vi "conf FCC Main Worst Position Measurement.vi"(8 "error in (no error)":errorcluster, 11 "SA Measurement in":refnum<class "SA Measurement.lvclass">) -> (0 "error out":errorcluster, 3 "SA Measurement out":refnum<class "SA Measurement.lvclass">)   [LabVIEW 2023, in "Spectrum Analyzer.lvlib" / "SA Measurement.lvclass"]
uses:
  SA Measurement.lvclass
  TYPE DEFINITION/Keysight 9020A/TYPE Measurement Preset.ctl
  TYPE DEFINITION/TYPE RBW and VBW Select.ctl
  TYPE DEFINITION/TYPE Marker Auto Select.ctl
  TYPE DEFINITION/TYPE Marker Control Mode.ctl
  SA Measurement.lvclass/SA Measurement.ctl
  Interface_Spectrum/Interface_Spectrum.lvclass
  Spectrum Analyzer.lvlib
  TYPE DEFINITION/TYPE Sweep Type Select.ctl
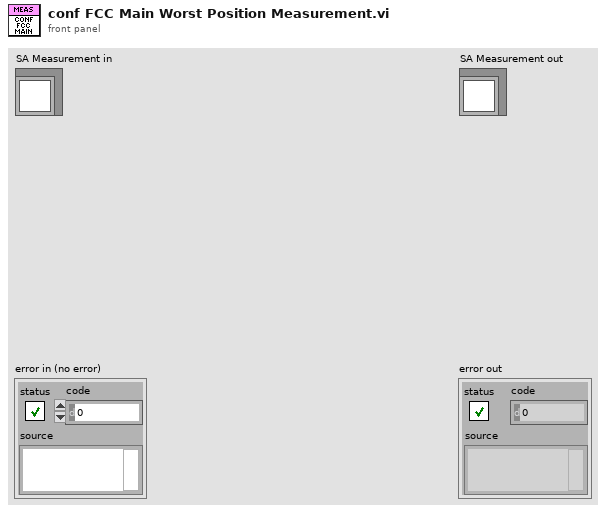
[diagram p1: front panel]
types:
  T1 = typedef "Spectrum Analyzer.lvlib/TYPE Sweep Type Select.ctl" = enum16{"Auto", "Sweep", "FFT"}
  T2 = typedef "Spectrum Analyzer.lvlib/TYPE Marker Control Mode.ctl" = enum16{"Normal", "Delta", "Off"}
  T3 = typedef "Spectrum Analyzer.lvlib/TYPE Marker Auto Select.ctl" = enum16{"Max Search Auto", "Min Search Auto"}
  T4 = typedef "Spectrum Analyzer.lvlib/TYPE RBW and VBW Select.ctl" = enum16{"Res BW", "Video BW"}
  T5 = typedef "Spectrum Analyzer.lvlib/TYPE Measurement Preset.ctl" = enum16{"Sweep SA Mode", "Channel Power", "Occupied BW", "ACP", "Spurious Emission", "Spurious Emission Mask", "Burst Power (Transmit Power)"}
  T6 = typedef "Spectrum Analyzer.lvlib/TYPE Y-axis Unit.ctl" = enum16{"dBm", "dBmV", "dBuV", "dBpW", "Volt", "Ampere", "Watt"}
  T7 = typedef "Spectrum Analyzer.lvlib/TYPE Reference Level and Atten Param.ctl" = cluster{"Reference Level":dbl, "Atten":i32, "Atten Auto?":bool, "Reference Level Offset":dbl}
  T8 = typedef "Spectrum Analyzer.lvlib/TYPE Display Trace Mode Select.ctl" = enum16{"Clear Write", "Max Hold", "Min Hold", "Average", "View"}
  T9 = typedef "Spectrum Analyzer.lvlib/TYPE Detect Mode Select.ctl" = enum16{"Det Auto (Normal)", "Auto Peak", "Positive Peak", "Negative Peak", "Sample", "RMS", "Average", "Quasipeak", "CISPR Average", "RMS Average"}
  T10 = cluster{"Trace Mode":T8, "Detector Type":T9, "Detect Auto?":bool}[]
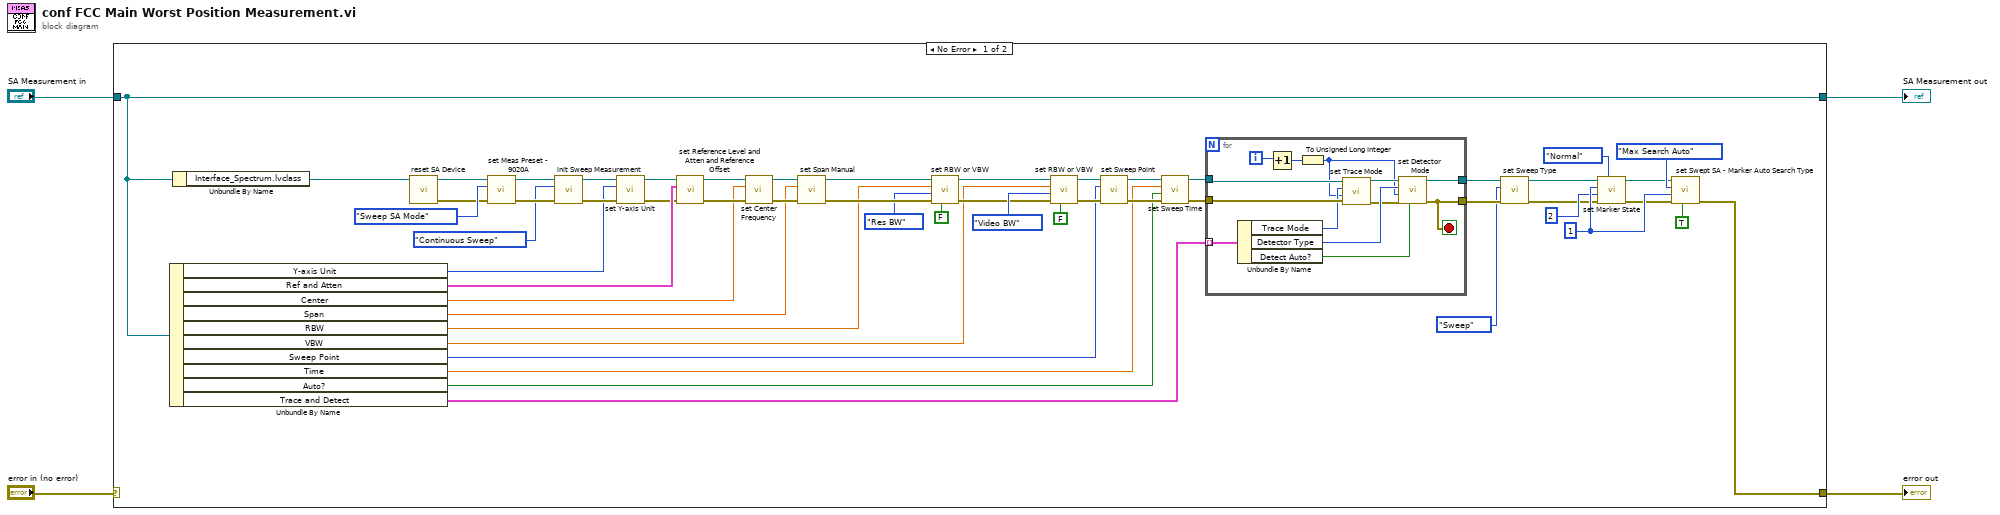
[diagram p0: block diagram]
diagram:
  n1 = case shown="No Error" "error in (no error)" {
    selector: "error in (no error)" -> [_ w72]
    tunnel: [w10 w72] -> w1
    tunnel: [w21 w71] -> w2
    tunnel: "SA Measurement in" -> [w21 w71]
    frame No Error {
      w14 = 1 ("Index")
      n2 = Unbundle By Name(w21) -> ("Y-axis Unit"=w32:T6, "Ref and Atten"=w53:T7, "Center"=w50:dbl, "Span"=w47:dbl, "RBW"=w44:dbl, "VBW"=w37:dbl, "Sweep Point"=w29:u32, "Time"=w26:dbl, "Auto?"=w25:bool, "Trace and Detect"=w22:T10)
      n3 = Unbundle By Name(w21) -> ("Interface_Spectrum.lvclass"=w20:refnum<class "Interface_Spectrum.lvclass">)
      n4 = call-dynamic "reset SA Device.vi"("Interface_Spectrum in"=w20) -> ("error out"=w18:errorcluster, "Interface_Spectrum out"=w19:refnum<class "Interface_Spectrum.lvclass">)  [unwired: 9 in]
      n5 = call-dynamic "set Meas Preset - 9020A.vi"("error in (no error)"=w18, "Measurement Preset"=TYPE_Measurement_Preset."Sweep SA Mode", "Interface_Spectrum in"=w19) -> ("error out"=w55:errorcluster, "Interface_Spectrum out"=w56:refnum<class "Interface_Spectrum.lvclass">)  [unwired: 7 in]
      n6 = call-dynamic "init Sweep Measurement.vi"("error in (no error)"=w55, "Sweep Measurement Mode"=enum16{"Single Sweep", "Continuous Sweep"}."Continuous Sweep", "Interface_Spectrum in"=w56) -> ("error out"=w35:errorcluster, "Interface_Spectrum out"=w36:refnum<class "Interface_Spectrum.lvclass">)  [unwired: 7 in]
      n7 = call-dynamic "set Y-axis Unit.vi"("error in (no error)"=w35, "Y-axis Unit"=w32, "Interface_Spectrum in"=w36) -> ("error out"=w33:errorcluster, "Interface_Spectrum out"=w34:refnum<class "Interface_Spectrum.lvclass">)  [unwired: 7 in]
      n8 = call-dynamic "set Reference Level and Atten and Reference Offset.vi"("error in (no error)"=w33, "Reference Level, Atten, Reference Offset"=w53, "Interface_Spectrum in"=w34) -> ("error out"=w51:errorcluster, "Interface_Spectrum out"=w52:refnum<class "Interface_Spectrum.lvclass">)  [unwired: 7 in]
      n9 = call-dynamic "set Center Frequency.vi"("error in (no error)"=w51, "Center Frequency (Hz)"=w50, "Interface_Spectrum in"=w52) -> ("error out"=w48:errorcluster, "Interface_Spectrum out"=w49:refnum<class "Interface_Spectrum.lvclass">)  [unwired: 7 in]
      n10 = call-dynamic "set Span Manual.vi"("error in (no error)"=w48, "Span (Hz)"=w47, "Interface_Spectrum in"=w49) -> ("error out"=w45:errorcluster, "Interface_Spectrum out"=w46:refnum<class "Interface_Spectrum.lvclass">)  [unwired: 7 in]
      n11 = call-dynamic "set RBW or VBW.vi"("BW Auto?"=FALSE, "error in (no error)"=w45, "BW Type"=TYPE_RBW_and_VBW_Select."Res BW", "BW Value (Hz)"=w44, "Interface_Spectrum in"=w46) -> ("error out"=w38:errorcluster, "Interface_Spectrum out"=w39:refnum<class "Interface_Spectrum.lvclass">)  [unwired: 5 in]
      n12 = call-dynamic "set RBW or VBW.vi"("BW Auto?"=FALSE, "error in (no error)"=w38, "BW Type"=TYPE_RBW_and_VBW_Select."Video BW", "BW Value (Hz)"=w37, "Interface_Spectrum in"=w39) -> ("error out"=w30:errorcluster, "Interface_Spectrum out"=w31:refnum<class "Interface_Spectrum.lvclass">)  [unwired: 5 in]
      n13 = call-dynamic "set Sweep Point.vi"("error in (no error)"=w30, "Sweep Point"=w29, "Interface_Spectrum in"=w31) -> ("error out"=w27:errorcluster, "Interface_Spectrum out"=w28:refnum<class "Interface_Spectrum.lvclass">)  [unwired: 7 in]
      n14 = call-dynamic "set Sweep Time.vi"("error in (no error)"=w27, "Sweep Time Auto?"=w25, "Sweep Time(sec)"=w26, "Interface_Spectrum in"=w28) -> ("error out"=w23:errorcluster, "Interface_Spectrum out"=w24:refnum<class "Interface_Spectrum.lvclass">)  [unwired: 6 in]
      n15 = for {
        tunnel: w24 -> [w69]
        tunnel: w23 -> [w68]
        tunnel: w22 -> [w70] mode=indexing
        tunnel: [w58] -> w8
        tunnel: [w59] -> w9
        i -> [w67]
        stop <- w58 stop-if-true
        n16 = Unbundle By Name(w70) -> ("Trace Mode"=w65:T8, "Detector Type"=w63:T9, "Detect Auto?"=w60:bool)
        n17 = Increment(x=w67) -> (x+1=w66:i32)
        n18 = To Unsigned Long Integer(number=w66) -> (unsigned 32bit integer=w61:u32)
        n19 = call-dynamic "set Trace Mode.vi"("error in (no error)"=w68, "Trace Index"=w61, "Trace Mode"=w65, "Interface_Spectrum in"=w69) -> ("error out"=w62:errorcluster, "Interface_Spectrum out"=w64:refnum<class "Interface_Spectrum.lvclass">)  [unwired: 6 in]
        n20 = call-dynamic "set Detector Mode.vi"("Detect Auto?"=w60, "error in (no error)"=w62, "Trace Index"=w61, "Detector Type"=w63, "Interface_Spectrum in"=w64) -> ("error out"=w58:errorcluster, "Interface_Spectrum out"=w59:refnum<class "Interface_Spectrum.lvclass">)  [unwired: 5 in]
      }
      n21 = call-dynamic "set Sweep Type.vi"("error in (no error)"=w8, "Sweep Mode"=TYPE_Sweep_Type_Select."Sweep", "Interface_Spectrum in"=w9) -> ("error out"=w6:errorcluster, "Interface_Spectrum out"=w7:refnum<class "Interface_Spectrum.lvclass">)  [unwired: 7 in]
      n22 = call-dynamic "set Marker State.vi"("Marker Mode"=TYPE_Marker_Control_Mode."Normal", "error in (no error)"=w6, "trace index"=2 ("Index"), "Marker Index"=w14, "Interface_Spectrum in"=w7) -> ("error out"=w11:errorcluster, "Interface_Spectrum out"=w12:refnum<class "Interface_Spectrum.lvclass">)  [unwired: 5 in]
      n23 = call-dynamic "set Swept SA - Marker Auto Search Type.vi"("Auto Search On?"=TRUE, "error in (no error)"=w11, "Index"=w14, "Marker Auto Type"=TYPE_Marker_Auto_Select."Max Search Auto", "Interface_Spectrum in"=w12) -> ("error out"=w10:errorcluster)  [unwired: 5 in, 1 out]
    }
    frame Error {
    }
  }
  "error out" <- w1
  "SA Measurement out" <- w2
